vi "PicoScope6000aGetTimebase2.vi"(4 "Number of Samples":u64, 6 "Memory Segment":u64, 7 "Acquisition Settings":T1={"preTriggerSamples"=0, "postTriggerSamples"=1000, "timebase"=2} {"postTriggerSamples" format="%_6p"; "preTriggerSamples" format="%_6p"}, 8 "error in (no error)":errorcluster, 11 "handle in":i16) -> (0 "error out":errorcluster, 3 "handle out":i16, 5 "Properties Panel":T2 {"Max Total Capture Time Available (sec)" format="%.3p"; "Sample Frequency" format="%.6p"; "Sample Rate" format="%.3p"; "Max Samples Available" format="%_6p"; "Total Capture Time (sec)" format="%.3p"})   [LabVIEW 2010]
doc: "Calls Gettimebase function"
uses:
  ps6000a.dll
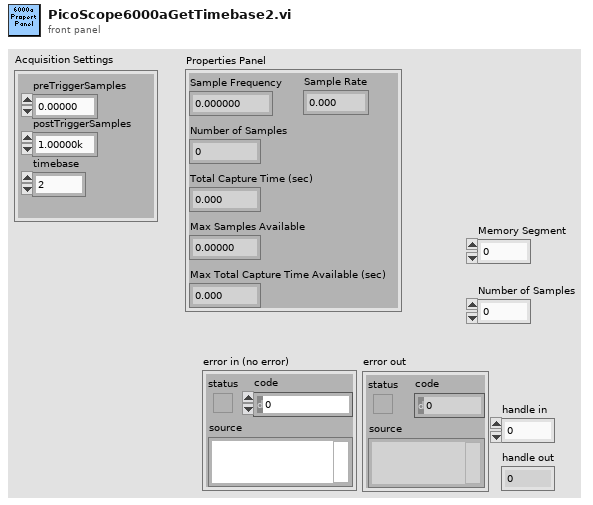
[diagram p1: front panel]
types:
  T1 = cluster{"preTriggerSamples":u64, "postTriggerSamples":u64, "timebase":u32}
  T2 = cluster{"Sample Frequency":dbl, "Sample Rate":dbl, "Max Samples Available":u64, "Number of Samples":u64, "Total Capture Time (sec) ":dbl, "Max Total Capture Time Available (sec)":dbl}
  T3 = cluster{sgl, sgl, "maxSamples":i32, "Number of Samples":u32, sgl, sgl}
  T4 = cluster{"status":bool, "code":u32, "source":string}
  T5 = cluster{dbl, dbl, "maxSamples":u64, "Number of Samples":u64, dbl, dbl}
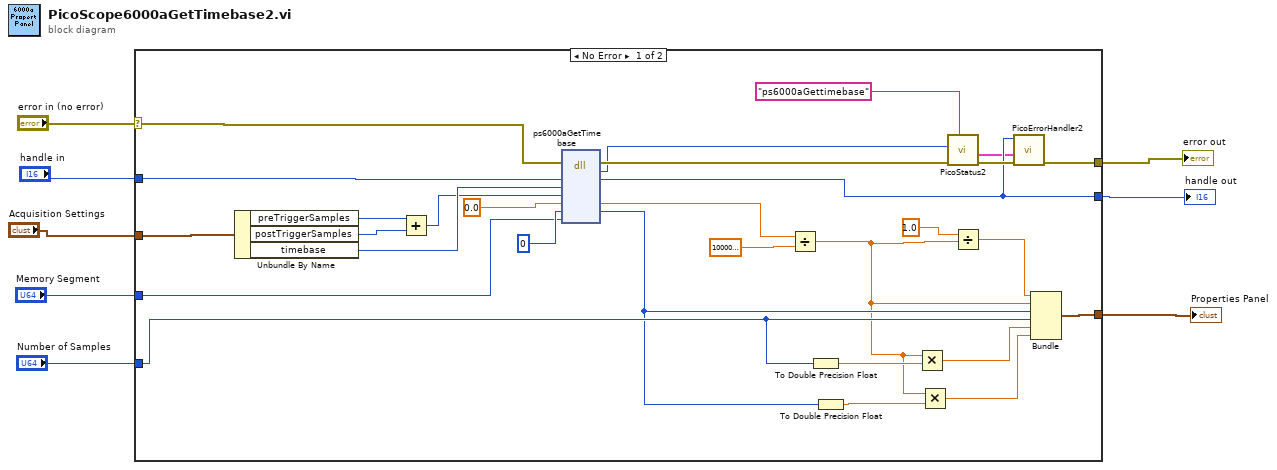
[diagram p0: block diagram]
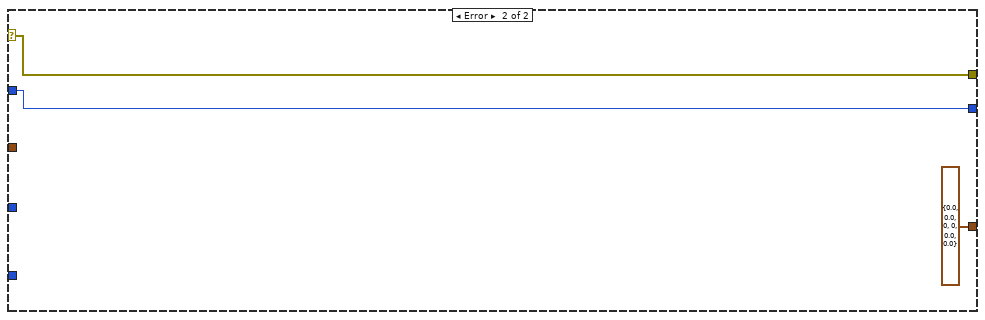
[diagram p2: hidden frame]
diagram:
  n1 = case shown="No Error" "error in (no error)" {
    selector: "error in (no error)" -> [w13 w40]
    tunnel: [w11 w40] -> w8
    tunnel: [w10 w39] -> w7
    tunnel: "Memory Segment" -> [w27 _]
    tunnel: "Number of Samples" -> [w21 _]
    tunnel: "handle in" -> [w26 w39]
    tunnel: "Acquisition Settings" -> [w25 _]
    tunnel: [w17 T3 {0.0, 0.0, "maxSamples"=0, "Number of Samples"=0, 0.0, 0.0}] -> w2
    frame No Error {
      n2 = Unbundle By Name(w25) -> ("preTriggerSamples"=w32:u64, "postTriggerSamples"=w33:u64, "timebase"=w34:u32)
      n3 = Add(x=w32, y=w33) -> (x+y=w23:u64)
      n4 = dll-call lib="ps6000a.dll" fn="ps6000aGetTimebase"(error in=w13, "handle"=w26, "timebase"=w34, "noSamples"=w23, "timeIntervalNanoseconds"=0.0, "maxSamples"=u64 0, "segmentIndex"=w27) -> (error out=w35:errorcluster, "PICO_STATUS"=w28:u32, "handle"=w10:i16, "timeIntervalNanoseconds"=w36:dbl, "maxSamples"=w19:u64)  [unwired: 5 in, 1 out]
      n5 = Divide(x=w36, y=1000000000.0) -> (x/y=w16:dbl)
      n6 = To Double Precision Float(number=w21) -> (double precision float=w24:dbl)
      n7 = To Double Precision Float(number=w19) -> (double precision float=w20:dbl)
      n8 = Multiply(x=w16, y=w24) -> (x*y=w22:dbl)
      n9 = Multiply(x=w16, y=w20) -> (x*y=w18:dbl)
      n10 = call "PicoStatus2.vi"("PICO source"="ps6000aGettimebase" ("source"), "Error in"=w35, "PICO STATUS"=w28) -> ("error out"=w12:errorcluster, "PICO_STATUS out"=w9:T4)  [unwired: 5 in]
      n11 = Divide(x=1.0, y=w16) -> (x/y=w14:dbl)
      n12 = call "PicoErrorHandler2.vi"("error in (no error)"=w12, "PICO_STATUS in"=w9, "handle In"=w10) -> ("error out"=w11:errorcluster)  [unwired: 8 in]
      n13 = Bundle(w14, w16, "maxSamples"=w19, "Number of Samples"=w21, w22, w18) -> (w17:T5)  [unwired: 1 in]
    }
    frame Error {
    }
  }
  "error out" <- w8
  "handle out" <- w7
  "Properties Panel" <- w2
